vi "Enqueue Request Message.vi"(5 "Request Callback":refnum<class "Callback.lvclass">, 6 "error in (no error)":errorcluster, 7 "Message Data":variant, 8 "Message":string, 9 "Process In":refnum<class "Process.lvclass">) -> (0 "error out":errorcluster, 3 "Process Out":refnum<class "Process.lvclass">)   [LabVIEW 2020]
doc: "For a regular message, enqueue the message. For a priority message, enqueue it at the front of the queue."
uses:
  Process.lvclass
  Callback/Callback.lvclass
  Process.lvclass/Process.ctl
  Protected/Messaging/Message Cluster.ctl
  C:/git/astemes-triarc-framework/source/Framework/Base/Base.lvclass
  C:/git/astemes-triarc-framework/source/Framework/Process/Process.lvclass
  C:/git/astemes-triarc-framework/source/Framework/Error Handler Interface/Error Handler Interface.lvclass
  C:/git/astemes-triarc-framework/source/Framework/Logging/Logging.lvclass
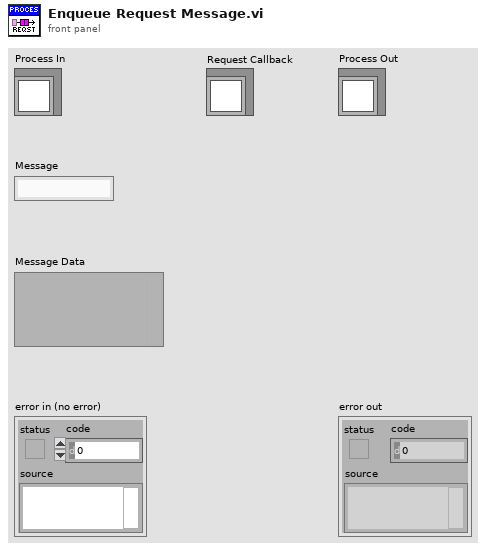
[diagram p1: front panel]
types:
  T1 = typedef "Process.lvclass/Message Cluster.ctl" = cluster{"Message":string, "Message Data":variant, "Request Callback":refnum<class "Callback.lvclass">}
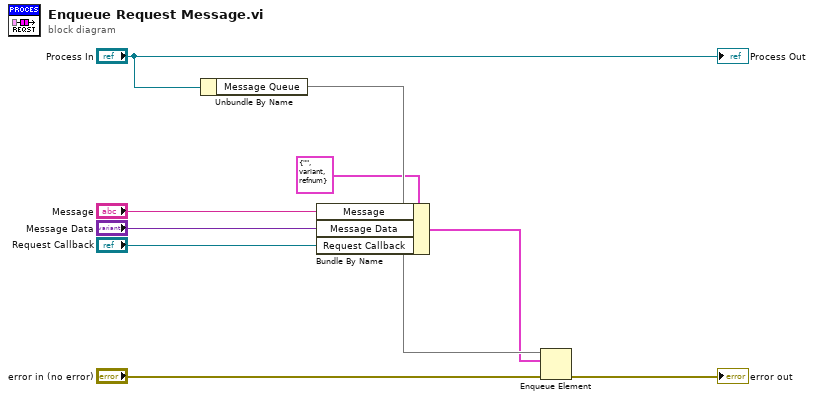
[diagram p0: block diagram]
diagram:
  n1 = Unbundle By Name("Process In") -> ("Message Queue"=w4)
  n2 = Bundle By Name(cluster=T1 {"Message"="", "Message Data"=variant, "Request Callback"=refnum} ("Message Cluster"), "Message"="Message", "Message Data"="Message Data", "Request Callback"="Request Callback") -> (w3:T1)
  n3 = Enqueue Element(queue=w4, element=w3, error in (no error)="error in (no error)") -> (error out=→"error out":errorcluster)  [unwired: 1 in, 2 out]
  "Process Out" <- "Process In"
